vi "test tools list title annotations.vi"(8 "error in (no error)":errorcluster) -> (0 "error out":errorcluster, 3 "body":string)   [LabVIEW 2020, in "MCP Server tests.lvlib"]
doc: "tools/list sends the optional title and annotations of a tool. fake_tool_annotated is registered with the title Annotated Fixture Tool and with readOnlyHint true and destructiveHint false, the other two hints not set: its entry must have that title and annotations with exactly those two keys. fake_tool_add is registered without title and annotations, so its entry has neither key. The request is sent with the LabVIEW HTTP Client directly."
uses:
  MCP Server tests.lvlib
  cdcbdaf3-3ee4-471c-bec7-a48854ea946e.vi
  853e2794-f4ae-4822-852b-1e4fcbe12919.vi
  <vilib>/JDP Science/JSONtext/Next JSON Value.vi
  <vilib>/JDP Science/JSONtext/String Subset.vi
  <vilib>/JDP Science/JSONtext/Parsing/Advance past next JSON Value (inlined COPY).vi
  <vilib>/JDP Science/JSONtext/Parsing/Advance past whitespace.vi
  <vilib>/JDP Science/JSONtext/Parsing/Advance past String.vi
  <vilib>/JDP Science/JSONtext/Parsing/Advance past Number.vi
  <vilib>/JDP Science/JSONtext/Parsing/Advance past Line Ending.vi
  <vilib>/JDP Science/JSONtext/Parsing/Parse Full Path or Item Name.vi
  <vilib>/JDP Science/JSONtext/Parsing/Advance past Array.vi
  <vilib>/JDP Science/JSONtext/Parsing/Advance past Object.vi
  <vilib>/JDP Science/JSONtext/support/Error Cluster From Code.vi
  <vilib>/JDP Science/JSONtext/Offset/Find Item Locations by Path.vi
  <vilib>/JDP Science/JSONtext/JSON text to Variant.vi
  <vilib>/JDP Science/JSONtext/LVClass Serializer/JSONtext LVClass Serializer.lvclass
  <vilib>/addons/_JKI Toolkits/Caraya/classes/Test/Test.lvclass
  <vilib>/JDP Science/JSONtext/JSONtext.lvlib
  <vilib>/addons/_JKI Toolkits/Caraya/classes/Assert/Assert.lvclass
panel:
  out "lookup error":errorcluster
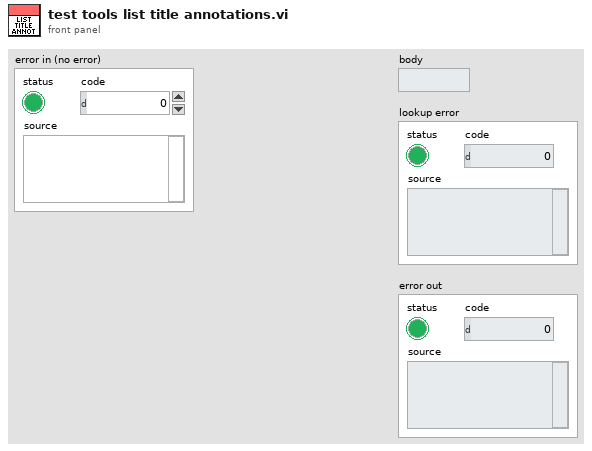
[diagram p1: front panel]
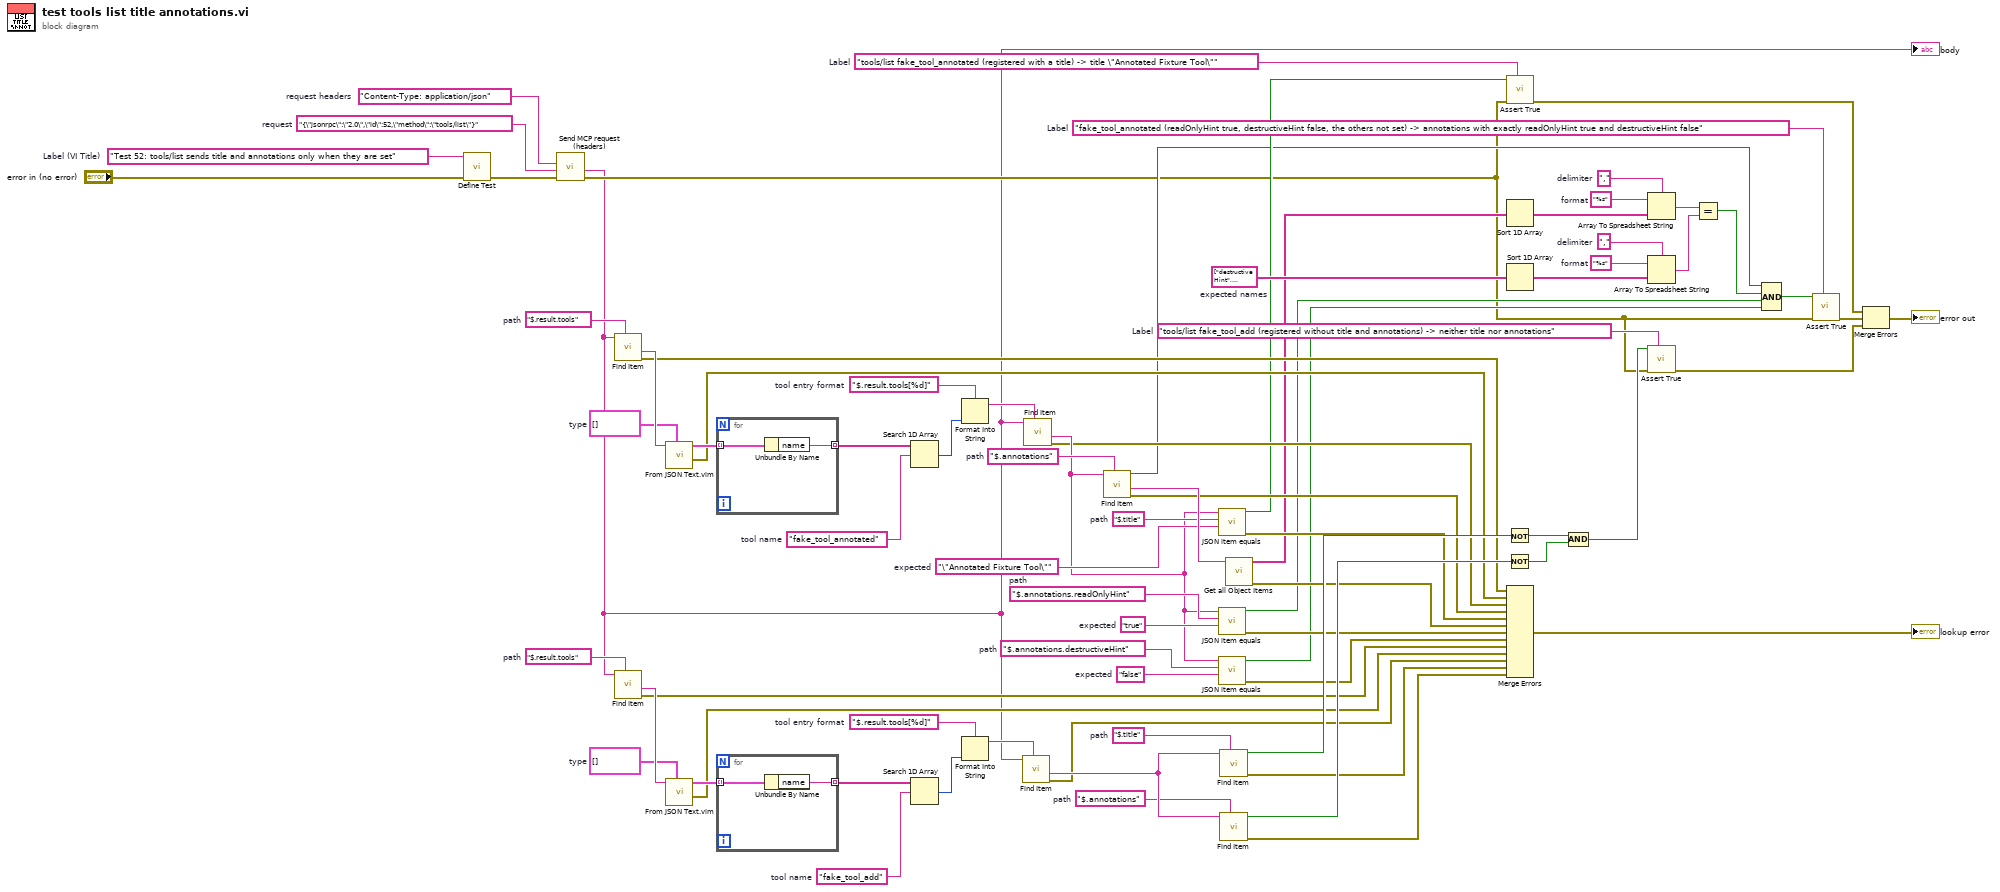
[diagram p0: block diagram]
diagram:
  w73 = "Content-Type: application/json"  # request headers
  w16 = "tools/list fake_tool_add (registered without title and annotations) -> neither title nor annotations"  # Label
  w7 = "fake_tool_annotated (readOnlyHint true, destructiveHint false, the others not set) -> annotations with exactly readOnlyHint true and destructiveHint false"  # Label
  w23 = "tools/list fake_tool_annotated (registered with a title) -> title \"Annotated Fixture Tool\""  # Label
  w49 = "$.annotations"  # path
  w51 = "$.title"  # path
  w55 = "$.result.tools[%d]"  # tool entry format
  w59 = "fake_tool_add"  # tool name
  w65 = cluster{"name":string}[] []  # type
  w69 = "$.result.tools"  # path
  w41 = "false"  # expected
  w42 = "$.annotations.destructiveHint"  # path
  w44 = "true"  # expected
  w45 = "$.annotations.readOnlyHint"  # path
  w74 = ","  # delimiter
  w76 = "%s"  # format
  w77 = string[] ["destructiveHint", "readOnlyHint"]  # expected names
  w18 = ","  # delimiter
  w20 = "%s"  # format
  w46 = "\"Annotated Fixture Tool\""  # expected
  w47 = "$.title"  # path
  w52 = "$.annotations"  # path
  w57 = "$.result.tools[%d]"  # tool entry format
  w61 = "fake_tool_annotated"  # tool name
  w67 = cluster{"name":string}[] []  # type
  w70 = "$.result.tools"  # path
  w72 = "{\"jsonrpc\":\"2.0\",\"id\":52,\"method\":\"tools/list\"}"  # request
  w79 = "Test 52: tools/list sends title and annotations only when they are set"  # Label (VI Title)
  n1 = call <vilib>:"Define Test.vi"("error in (no error)"="error in (no error)", "Label (VI Title)"=w79) -> ("error out"=w71:errorcluster)  [unwired: 8 in, 1 out]
  n2 = call "Send MCP request (headers).vi"("error in (no error)"=w71, "request"=w72, "request headers"=w73) -> ("error out"=w8:errorcluster, "response"=w3:string)  [unwired: 5 in, 2 out]
  "body" <- w3
  n3 = call <vilib>:"Find Item.vi"("$Path or Item Name"=w70, "JSON"=w3) -> ("error out"=w38:errorcluster, "<JSON>"=w68:string)  [unwired: 6 in, 2 out]
  n4 = call <vilib>:"Find Item.vi"("$Path or Item Name"=w69, "JSON"=w3) -> ("error out"=w30:errorcluster, "<JSON>"=w66:string)  [unwired: 6 in, 2 out]
  n5 = call "From JSON Text.vim"("Data Type and Default Value"=w67, "JSON"=w68) -> ("error out"=w37:errorcluster, "Data out"=w64:cluster{"name":string}[])  [unwired: 8 in]
  n6 = call "From JSON Text.vim"("Data Type and Default Value"=w65, "JSON"=w66) -> ("error out"=w29:errorcluster, "Data out"=w63:cluster{"name":string}[])  [unwired: 8 in]
  n7 = for {
    tunnel: w64 -> [w81] mode=indexing
    tunnel: [w80] -> w62 mode=indexing
    n8 = Unbundle By Name(w81) -> ("name"=w80:string)
  }
  n9 = for {
    tunnel: w63 -> [w83] mode=indexing
    tunnel: [w82] -> w60 mode=indexing
    n10 = Unbundle By Name(w83) -> ("name"=w82:string)
  }
  n11 = Search 1D Array(1D array=w62, element=w61) -> (index of element=w58:i32)  [unwired: 1 in]
  n12 = Search 1D Array(1D array=w60, element=w59) -> (index of element=w56:i32)  [unwired: 1 in]
  n13 = Format Into String(format string=w57, w58) -> (resulting string=w54:string)  [unwired: 2 in, 1 out]
  n14 = Format Into String(format string=w55, w56) -> (resulting string=w53:string)  [unwired: 2 in, 1 out]
  n15 = call <vilib>:"Find Item.vi"("$Path or Item Name"=w53, "JSON"=w3) -> ("error out"=w28:errorcluster, "<JSON>"=w50:string)  [unwired: 6 in, 2 out]
  n16 = call <vilib>:"Find Item.vi"("$Path or Item Name"=w54, "JSON"=w3) -> ("error out"=w36:errorcluster, "<JSON>"=w43:string)  [unwired: 6 in, 2 out]
  n17 = call <vilib>:"Find Item.vi"("$Path or Item Name"=w52, "JSON"=w43) -> ("error out"=w35:errorcluster, "<JSON>"=w48:string, "Found"=w13:bool)  [unwired: 6 in, 1 out]
  n18 = call "JSON item equals.vi"("expected"=w46, "path"=w47, "JSON"=w43) -> ("error out"=w34:errorcluster, "equal?"=w24:bool)  [unwired: 6 in, 1 out]
  n19 = call "JSON item equals.vi"("expected"=w44, "path"=w45, "JSON"=w43) -> ("error out"=w32:errorcluster, "equal?"=w11:bool)  [unwired: 6 in, 1 out]
  n20 = call "JSON item equals.vi"("expected"=w41, "path"=w42, "JSON"=w43) -> ("error out"=w31:errorcluster, "equal?"=w10:bool)  [unwired: 6 in, 1 out]
  n21 = call <vilib>:"Find Item.vi"("$Path or Item Name"=w51, "JSON"=w50) -> ("error out"=w27:errorcluster, "Found"=w40:bool)  [unwired: 6 in, 2 out]
  n22 = call <vilib>:"Find Item.vi"("$Path or Item Name"=w49, "JSON"=w50) -> ("error out"=w26:errorcluster, "Found"=w39:bool)  [unwired: 6 in, 2 out]
  n23 = call <vilib>:"Get all Object Items.vi"("JSON"=w48) -> ("error out"=w33:errorcluster, "Item Names"=w25:string[])  [unwired: 7 in, 2 out]
  n24 = Not(x=w40) -> (.not. x?=w22:bool)
  n25 = Not(x=w39) -> (.not. x?=w21:bool)
  n26 = call <vilib>:"Assert True.vi"("Label"=w23, "error in (no error)"=w8, "True?"=w24) -> ("error out"=w6:errorcluster)  [unwired: 7 in, 1 out]
  n27 = Sort 1D Array(array=w25) -> (sorted array=w19:string[])
  n28 = Sort 1D Array(array=w77) -> (sorted array=w75:string[])
  n29 = Merge Errors(w38, w37, w36, w35, w34, w33, w32, w31, w30, w29, w28, w27, w26) -> (→"lookup error":errorcluster)
  n30 = Compound Arithmetic op=AND(w22, w21) -> (w17:bool)
  n31 = Array To Spreadsheet String(delimiter (Tab)=w18, array=w19, 3:w20) -> (spreadsheet string=w15:string)
  n32 = Array To Spreadsheet String(delimiter (Tab)=w74, array=w75, 3:w76) -> (spreadsheet string=w14:string)
  n33 = call <vilib>:"Assert True.vi"("Label"=w16, "error in (no error)"=w8, "True?"=w17) -> ("error out"=w4:errorcluster)  [unwired: 7 in, 1 out]
  n34 = Equal?(x=w15, y=w14) -> (x = y?=w12:bool)
  n35 = Compound Arithmetic op=AND(w13, w12, w11, w10) -> (w9:bool)
  n36 = call <vilib>:"Assert True.vi"("Label"=w7, "error in (no error)"=w8, "True?"=w9) -> ("error out"=w5:errorcluster)  [unwired: 7 in, 1 out]
  n37 = Merge Errors(w6, w5, w4) -> (→"error out":errorcluster)
